vi "DeleteGraph2.vi"(10 "StileIn":T1(array[cluster])=[{"Plot.Bar Plot Style"=0, "Plot.DigitalLineStyle"=1, "Plot.Line Style"=0, "Plot.Line Width"=2, "Plot.Plot Color"=5863167, "Plot.Plot Name"="Plot 0", "Plot.Point Style"=0}, {"Plot.Bar Plot Style"=0, "Plot.DigitalLineStyle"=1, "Plot.Line Style"=0, "Plot.Line Width"=2, "Plot.Plot Color"=13257796, "Plot.Plot Name"="Plot 1", "Plot.Point Style"=0}, {"Plot.Bar Plot Style"=0, "Plot.DigitalLineStyle"=1, "Plot.Line Style"=0, "Plot.Line Width"=2, "Plot.Plot Color"=6601816, "Plot.Plot Name"="Plot 2", "Plot.Point Style"=0}, {"Plot.Bar Plot Style"=0, "Plot.DigitalLineStyle"=1, "Plot.Line Style"=0, "Plot.Line Width"=2, "Plot.Plot Color"=15441725, "Plot.Plot Name"="Plot 3", "Plot.Point Style"=0}, {"Plot.Bar Plot Style"=0, "Plot.DigitalLineStyle"=1, "Plot.Line Style"=0, "Plot.Line Width"=2, "Plot.Plot Color"=8742822, "Plot.Plot Name"="Plot 4", "Plot.Point Style"=0}, {"Plot.Bar Plot Style"=0, "Plot.DigitalLineStyle"=1, "Plot.Line Style"=0, "Plot.Line Width"=3, "Plot.Plot Color"=10051840, "Plot.Plot Name"="Plot 5", "Plot.Point Style"=0}, {"Plot.Bar Plot Style"=0, "Plot.DigitalLineStyle"=1, "Plot.Line Style"=0, "Plot.Line Width"=3, "Plot.Plot Color"=3121844, "Plot.Plot Name"="Plot 6", "Plot.Point Style"=0}, {"Plot.Bar Plot Style"=0, "Plot.DigitalLineStyle"=1, "Plot.Line Style"=0, "Plot.Line Width"=3, "Plot.Plot Color"=13592771, "Plot.Plot Name"="Plot 7", "Plot.Point Style"=0}, {"Plot.Bar Plot Style"=0, "Plot.DigitalLineStyle"=1, "Plot.Line Style"=0, "Plot.Line Width"=3, "Plot.Plot Color"=931427, "Plot.Plot Name"="Plot 8", "Plot.Point Style"=0}, {"Plot.Bar Plot Style"=0, "Plot.DigitalLineStyle"=1, "Plot.Line Style"=0, "Plot.Line Width"=3, "Plot.Plot Color"=9014678, "Plot.Plot Name"="Plot 9", "Plot.Point Style"=0}, {"Plot.Bar Plot Style"=0, "Plot.DigitalLineStyle"=1, "Plot.Line Style"=0, "Plot.Line Width"=0, "Plot.Plot Color"=14483242, "Plot.Plot Name"="Plot 10", "Plot.Point Style"=0}, {"Plot.Bar Plot Style"=0, "Plot.DigitalLineStyle"=1, "Plot.Line Style"=0, "Plot.Line Width"=1, "Plot.Plot Color"=9538739, "Plot.Plot Name"="Plot 11", "Plot.Point Style"=0}, {"Plot.Bar Plot Style"=0, "Plot.DigitalLineStyle"=1, "Plot.Line Style"=0, "Plot.Line Width"=0, "Plot.Plot Color"=982784, "Plot.Plot Name"="Plot 12", "Plot.Point Style"=0}, {"Plot.Bar Plot Style"=0, "Plot.DigitalLineStyle"=1, "Plot.Line Style"=0, "Plot.Line Width"=0, "Plot.Plot Color"=4375295, "Plot.Plot Name"="Plot 13", "Plot.Point Style"=0}, {"Plot.Bar Plot Style"=0, "Plot.DigitalLineStyle"=1, "Plot.Line Style"=0, "Plot.Line Width"=0, "Plot.Plot Color"=13827953, "Plot.Plot Name"="Plot 14", "Plot.Point Style"=0}, {"Plot.Bar Plot Style"=0, "Plot.DigitalLineStyle"=1, "Plot.Line Style"=0, "Plot.Line Width"=0, "Plot.Plot Color"=13457919, "Plot.Plot Name"="Plot 15", "Plot.Point Style"=0}, {"Plot.Bar Plot Style"=0, "Plot.DigitalLineStyle"=1, "Plot.Line Style"=0, "Plot.Line Width"=0, "Plot.Plot Color"=16757522, "Plot.Plot Name"="Plot 16", "Plot.Point Style"=0}, {"Plot.Bar Plot Style"=0, "Plot.DigitalLineStyle"=1, "Plot.Line Style"=0, "Plot.Line Width"=0, "Plot.Plot Color"=4343295, "Plot.Plot Name"="Plot 17", "Plot.Point Style"=0}, {"Plot.Bar Plot Style"=0, "Plot.DigitalLineStyle"=1, "Plot.Line Style"=0, "Plot.Line Width"=0, "Plot.Plot Color"=16728758, "Plot.Plot Name"="Plot 18", "Plot.Point Style"=0}, {"Plot.Bar Plot Style"=0, "Plot.DigitalLineStyle"=1, "Plot.Line Style"=0, "Plot.Line Width"=0, "Plot.Plot Color"=5898228, "Plot.Plot Name"="Plot 19", "Plot.Point Style"=0}], 11 "GraphIN":T2) -> (2 "StileOUT":T1(array[cluster]), 3 "GraphOUT":T2)   [LabVIEW 2017]
uses:
  controls/st_str Graph Data.ctl
  <vilib>/Utility/miscctls.llb/LVAnnotationListTypeDef.ctl
  <vilib>/Utility/miscctls.llb/LVCursorListTypeDef.ctl
panel:
  out "Array Stile 2":T1(array[cluster])
  out "x+y":dbl
  out "Array StileSave":T1(array[cluster])
  out "error out":errorcluster
  in  "DeleteALLPlot":bool
  out "Array Stile":T1(array[cluster])=[{"Plot.Bar Plot Style"=0, "Plot.DigitalLineStyle"=1, "Plot.Line Style"=0, "Plot.Line Width"=3, "Plot.Plot Color"=3113143, "Plot.Plot Name"=" Plot 0", "Plot.Point Style"=0}, {"Plot.Bar Plot Style"=0, "Plot.DigitalLineStyle"=1, "Plot.Line Style"=0, "Plot.Line Width"=3, "Plot.Plot Color"=13257796, "Plot.Plot Name"=" Plot 1", "Plot.Point Style"=0}, {"Plot.Bar Plot Style"=0, "Plot.DigitalLineStyle"=1, "Plot.Line Style"=0, "Plot.Line Width"=3, "Plot.Plot Color"=6601816, "Plot.Plot Name"="Plot 2", "Plot.Point Style"=0}, {"Plot.Bar Plot Style"=0, "Plot.DigitalLineStyle"=1, "Plot.Line Style"=0, "Plot.Line Width"=3, "Plot.Plot Color"=15441725, "Plot.Plot Name"="Plot 3", "Plot.Point Style"=0}, {"Plot.Bar Plot Style"=0, "Plot.DigitalLineStyle"=1, "Plot.Line Style"=0, "Plot.Line Width"=3, "Plot.Plot Color"=8742822, "Plot.Plot Name"="Plot 4", "Plot.Point Style"=0}, {"Plot.Bar Plot Style"=0, "Plot.DigitalLineStyle"=1, "Plot.Line Style"=0, "Plot.Line Width"=3, "Plot.Plot Color"=10051840, "Plot.Plot Name"="Plot 5", "Plot.Point Style"=0}, {"Plot.Bar Plot Style"=0, "Plot.DigitalLineStyle"=1, "Plot.Line Style"=0, "Plot.Line Width"=3, "Plot.Plot Color"=3121844, "Plot.Plot Name"="Plot 6", "Plot.Point Style"=0}, {"Plot.Bar Plot Style"=0, "Plot.DigitalLineStyle"=1, "Plot.Line Style"=0, "Plot.Line Width"=3, "Plot.Plot Color"=13592771, "Plot.Plot Name"="Plot 7", "Plot.Point Style"=0}, {"Plot.Bar Plot Style"=0, "Plot.DigitalLineStyle"=1, "Plot.Line Style"=0, "Plot.Line Width"=3, "Plot.Plot Color"=931427, "Plot.Plot Name"="Plot 8", "Plot.Point Style"=0}, {"Plot.Bar Plot Style"=0, "Plot.DigitalLineStyle"=1, "Plot.Line Style"=0, "Plot.Line Width"=3, "Plot.Plot Color"=9014678, "Plot.Plot Name"="Plot 9", "Plot.Point Style"=0}, {"Plot.Bar Plot Style"=0, "Plot.DigitalLineStyle"=1, "Plot.Line Style"=0, "Plot.Line Width"=0, "Plot.Plot Color"=16777215, "Plot.Plot Name"="Plot 10", "Plot.Point Style"=0}, {"Plot.Bar Plot Style"=0, "Plot.DigitalLineStyle"=1, "Plot.Line Style"=0, "Plot.Line Width"=0, "Plot.Plot Color"=16728642, "Plot.Plot Name"="Plot11", "Plot.Point Style"=0}, {"Plot.Bar Plot Style"=0, "Plot.DigitalLineStyle"=1, "Plot.Line Style"=0, "Plot.Line Width"=0, "Plot.Plot Color"=982784, "Plot.Plot Name"="Plot 12", "Plot.Point Style"=0}, {"Plot.Bar Plot Style"=0, "Plot.DigitalLineStyle"=1, "Plot.Line Style"=0, "Plot.Line Width"=0, "Plot.Plot Color"=4375295, "Plot.Plot Name"="Plot 13", "Plot.Point Style"=0}, {"Plot.Bar Plot Style"=0, "Plot.DigitalLineStyle"=1, "Plot.Line Style"=0, "Plot.Line Width"=0, "Plot.Plot Color"=13827953, "Plot.Plot Name"="Plot 14", "Plot.Point Style"=0}, {"Plot.Bar Plot Style"=0, "Plot.DigitalLineStyle"=1, "Plot.Line Style"=0, "Plot.Line Width"=0, "Plot.Plot Color"=13457919, "Plot.Plot Name"="Plot 15", "Plot.Point Style"=0}, {"Plot.Bar Plot Style"=0, "Plot.DigitalLineStyle"=1, "Plot.Line Style"=0, "Plot.Line Width"=0, "Plot.Plot Color"=16757522, "Plot.Plot Name"="Plot 16", "Plot.Point Style"=0}, {"Plot.Bar Plot Style"=0, "Plot.DigitalLineStyle"=1, "Plot.Line Style"=0, "Plot.Line Width"=0, "Plot.Plot Color"=4343295, "Plot.Plot Name"="Plot 17", "Plot.Point Style"=0}, {"Plot.Bar Plot Style"=0, "Plot.DigitalLineStyle"=1, "Plot.Line Style"=0, "Plot.Line Width"=0, "Plot.Plot Color"=16728758, "Plot.Plot Name"="Plot 18", "Plot.Point Style"=0}, {"Plot.Bar Plot Style"=0, "Plot.DigitalLineStyle"=1, "Plot.Line Style"=0, "Plot.Line Width"=0, "Plot.Plot Color"=5898228, "Plot.Plot Name"="Plot 19", "Plot.Point Style"=0}, {"Plot.Bar Plot Style"=0, "Plot.DigitalLineStyle"=1, "Plot.Line Style"=0, "Plot.Line Width"=3, "Plot.Plot Color"=476624, "Plot.Plot Name"="Plot 20", "Plot.Point Style"=0}, {"Plot.Bar Plot Style"=0, "Plot.DigitalLineStyle"=1, "Plot.Line Style"=0, "Plot.Line Width"=3, "Plot.Plot Color"=411336, "Plot.Plot Name"="Plot 21", "Plot.Point Style"=0}]
  in  "DeleteSelectPlot":bool
  in  "Exit":bool
  out "АЧХIn":cluster{dbl[], dbl[]}[](graph)=[{[10.0], [0.9990420594251289]}, {[10.0, 20.0, 30.0, 40.0, 50.0, 60.0, 70.0, 80.0, 90.0, 100.0], [0.9990710865943554, 0.9983737368547715, 0.9976213766215998, 0.9969952678672057, 0.9967386681898875, 0.9967158758213325, 0.9966216633883461, 0.9967130281386235, 0.997241304832117, 0.9978171905888101]}, {[10.0, 20.0, 30.0, 40.0, 50.0, 60.0, 70.0, 80.0, 90.0, 100.0], [0.9988829040935796, 0.998316804468434, 0.9975357463328959, 0.9968238922918776, 0.9966331250389342, 0.9964782615048055, 0.9964769254923784, 0.9965780617245455, 0.9971895145348859, 0.9977820844166819]}, {[100.0, 110.0, 120.0, 130.0, 140.0, 150.0, 160.0, 170.0, 180.0, 190.0, 200.0], [0.9976024425934543, 0.9979153955951243, 0.9977501265851223, 0.9976091903479634, 0.997569296017074, 0.9976312638585361, 0.9976378149884235, 0.9975972662804196, 0.9976213719667596, 0.9977412021645674, 0.9978437042833532]}] caption="XY Graph - Light"
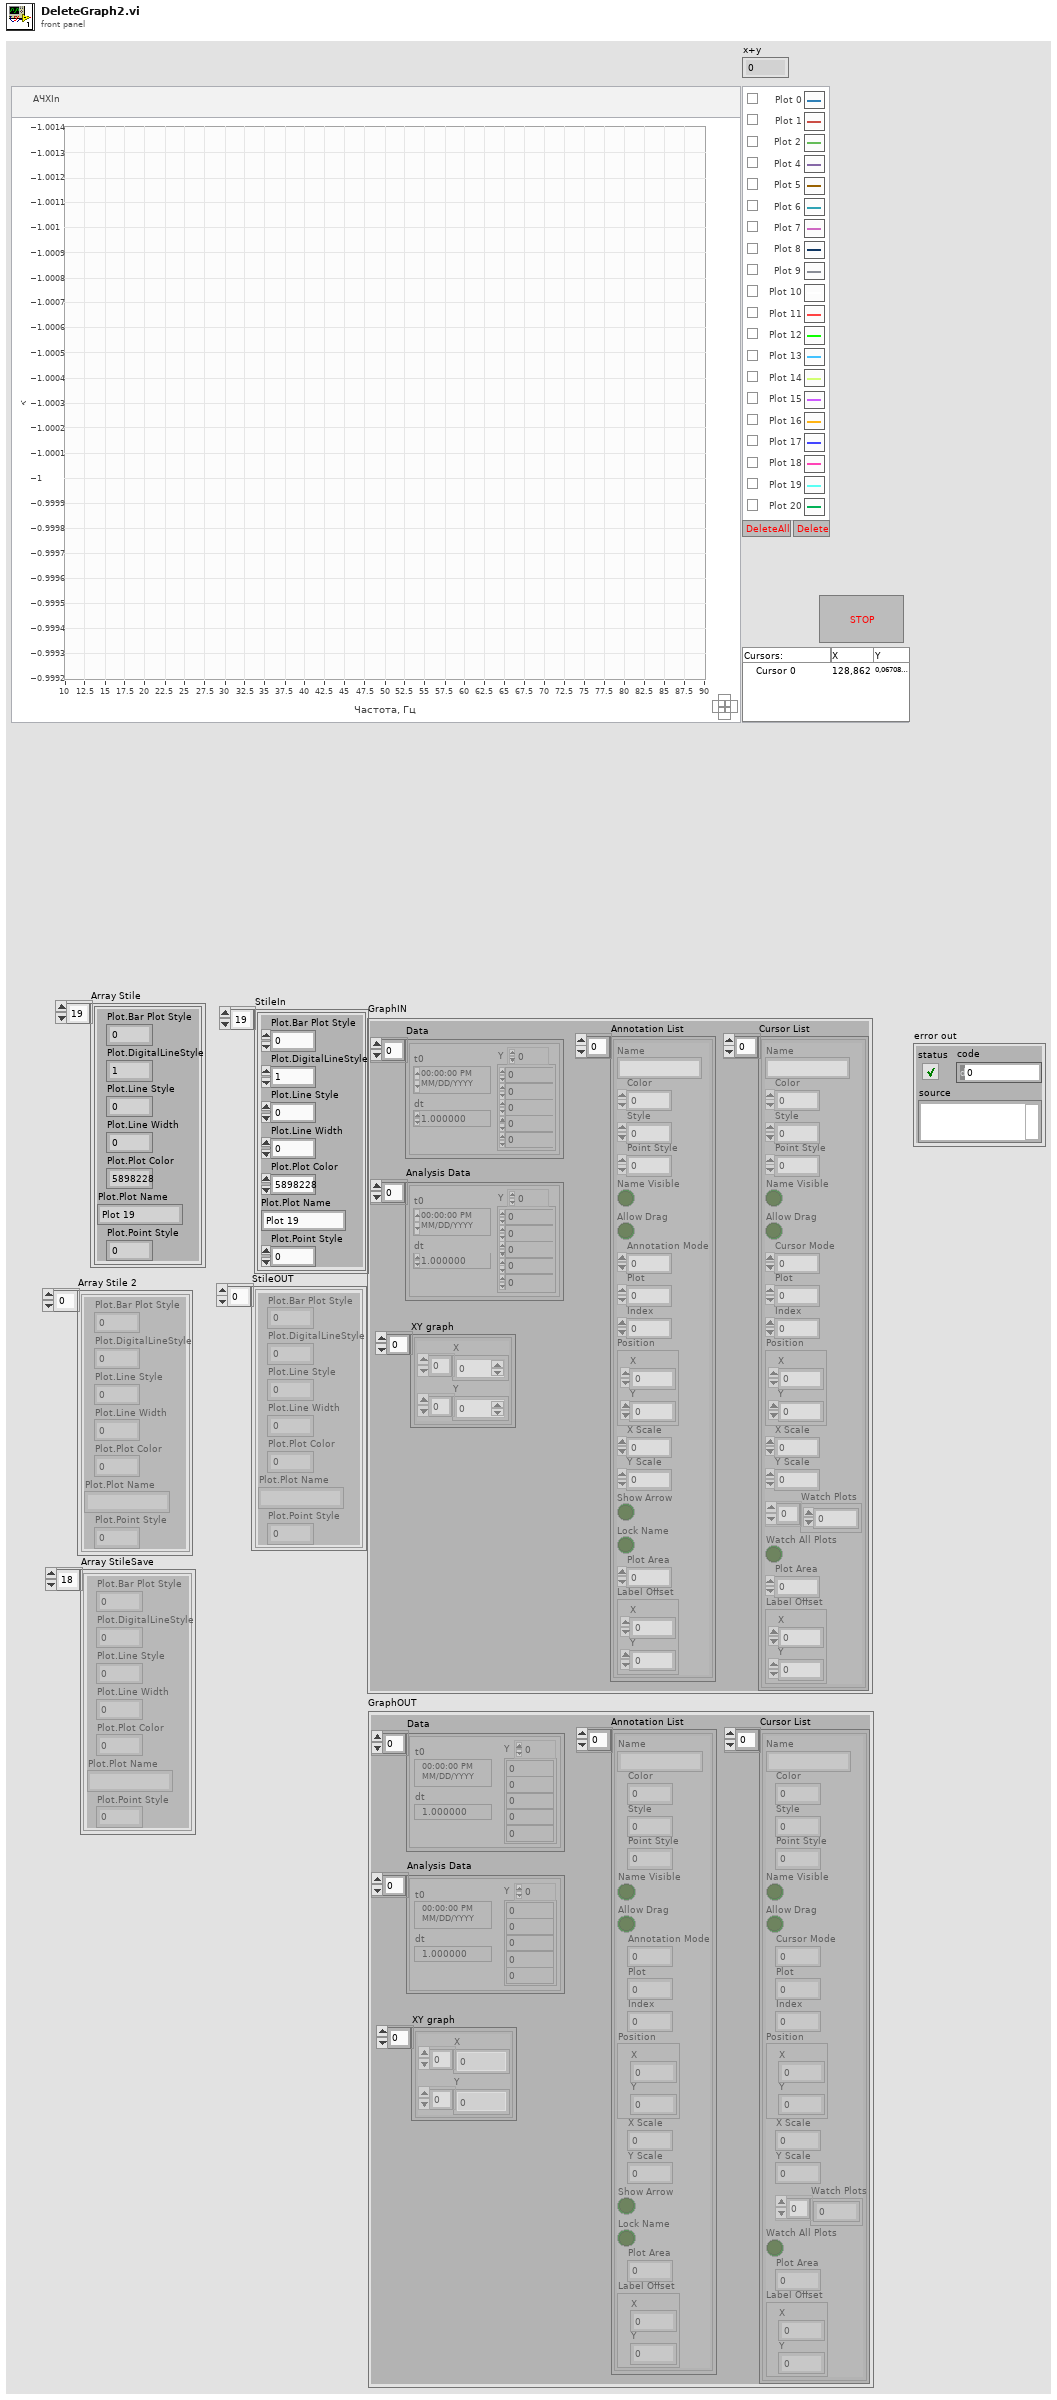
[diagram p1: front panel]
types:
  T1 = cluster{"Plot.Bar Plot Style":u8, "Plot.DigitalLineStyle":u8, "Plot.Line Style":u8, "Plot.Line Width":u8, "Plot.Plot Color":u32, "Plot.Plot Name":string, "Plot.Point Style":u8}[]
  T2 = typedef "st_str Graph Data.ctl" = cluster{"Data":waveform(dbl)[], "Annotation List":T3, "Cursor List":T4, "Analysis Data":waveform(dbl)[], "XY graph":cluster{"X":dbl[], "Y":dbl[]}[]}
  T3 = typedef "LVAnnotationListTypeDef.ctl" = cluster{"Name":string, "Color":u32, "Style":u8, "Point Style":u8, "Name Visible":bool, "Allow Drag":bool, "Annotation Mode":u32, "Plot":i32, "Index":i32, "Position":cluster{"X":dbl, "Y":dbl}, "X Scale":u32, "Y Scale":u32, "Show Arrow":bool, "Lock Name":bool, "Plot Area":i32, "Label Offset":cluster{"X":dbl, "Y":dbl}}[]
  T4 = typedef "LVCursorListTypeDef.ctl" = cluster{"Name":string, "Color":u32, "Style":u8, "Point Style":u8, "Name Visible":bool, "Allow Drag":bool, "Cursor Mode":u32, "Plot":i32, "Index":i32, "Position":cluster{"X":dbl, "Y":dbl}, "X Scale":u32, "Y Scale":u32, "Watch Plots":i32[], "Watch All Plots":bool, "Plot Area":i32, "Label Offset":cluster{"X":dbl, "Y":dbl}}[]
  T5 = cluster{"Plot.Bar Plot Style":u8, "Plot.DigitalLineStyle":u8, "Plot.Line Style":u8, "Plot.Line Width":u8, "Plot.Plot Color":u32, "Plot.Plot Name":string, "Plot.Point Style":u8}
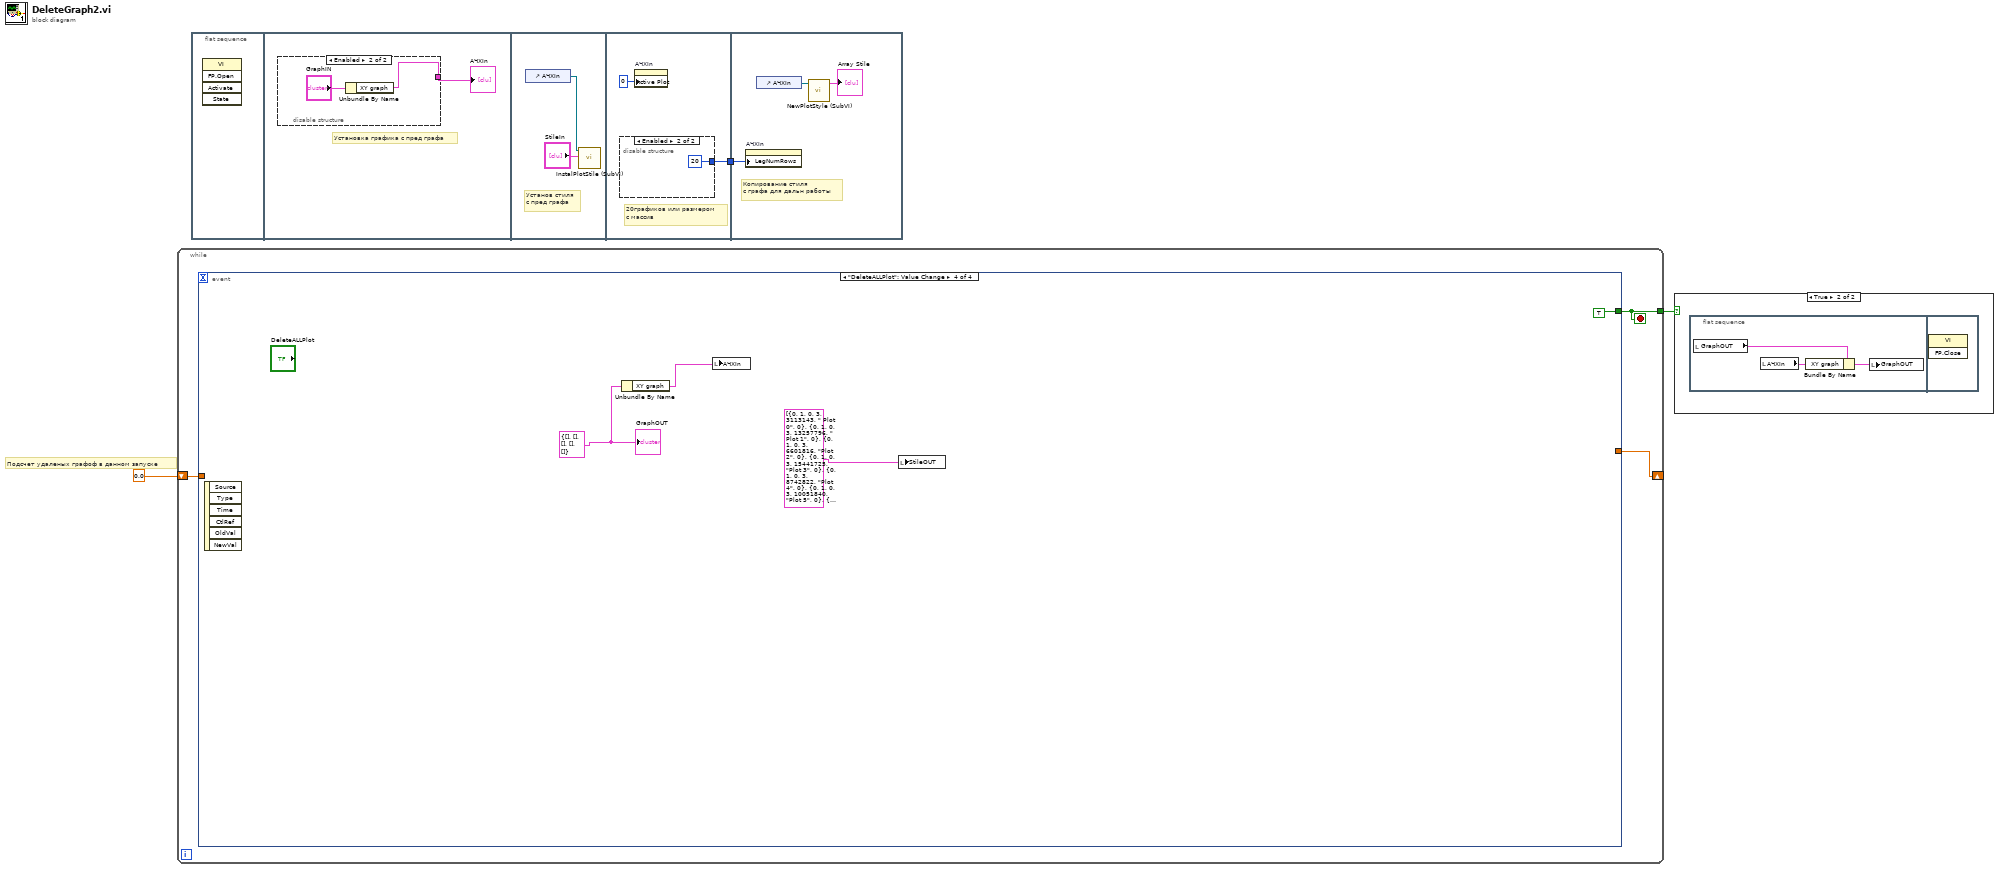
[diagram p0: block diagram]
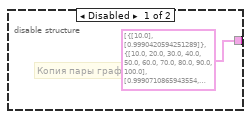
[diagram p3: hidden frame]
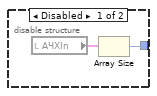
[diagram p4: hidden frame]
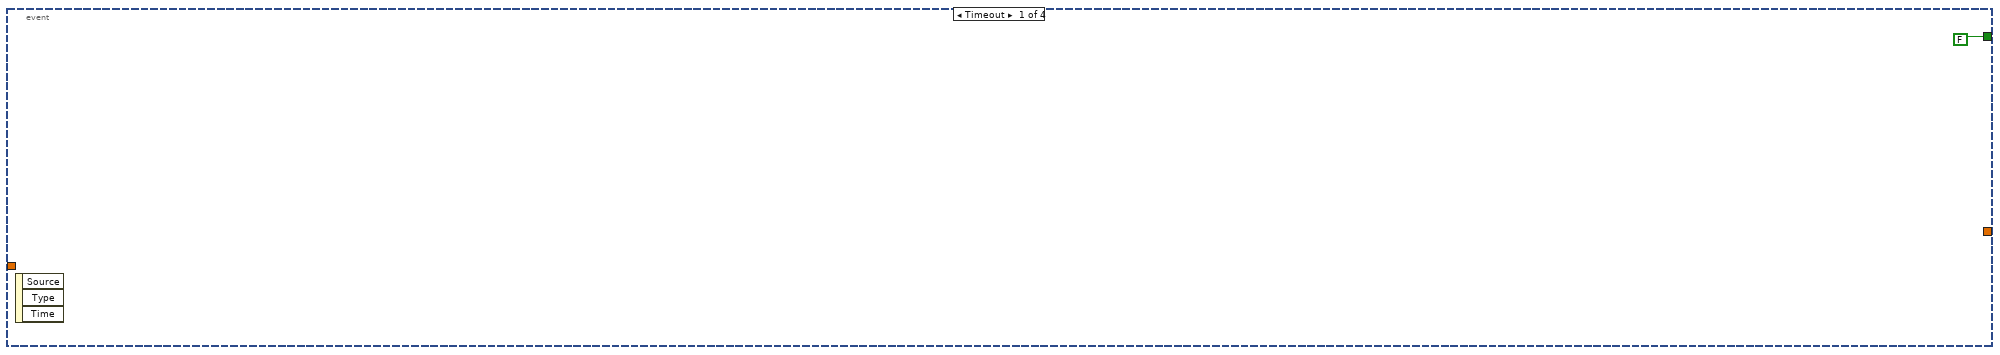
[diagram p5: hidden frame]
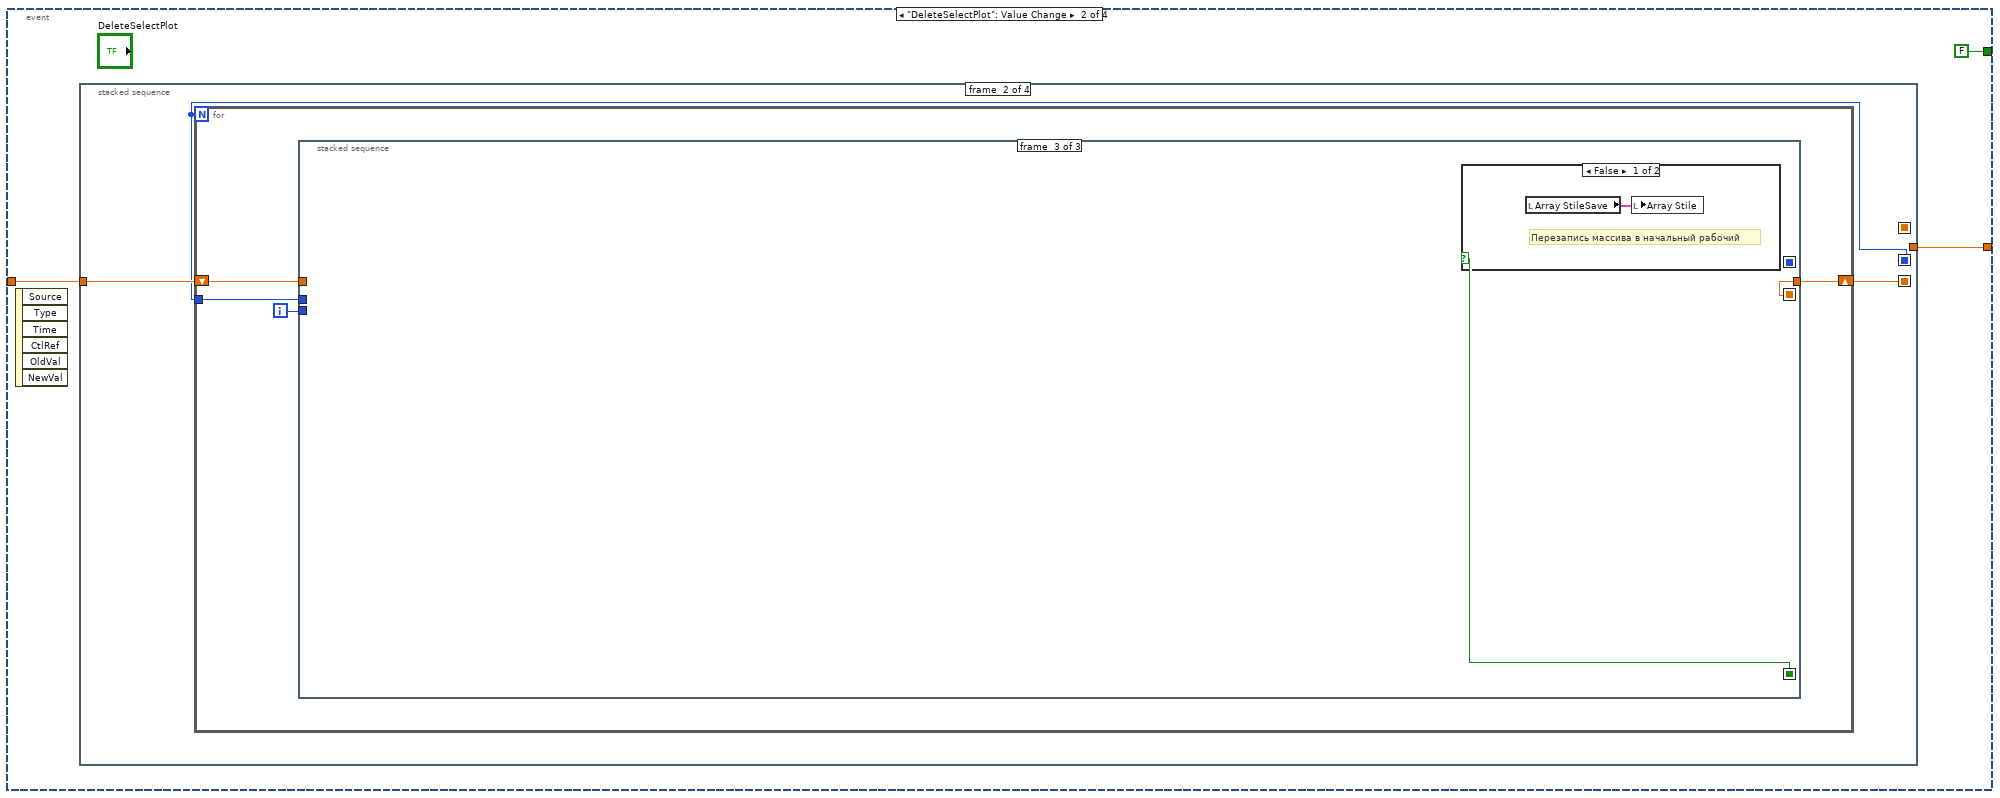
[diagram p6: hidden frame]
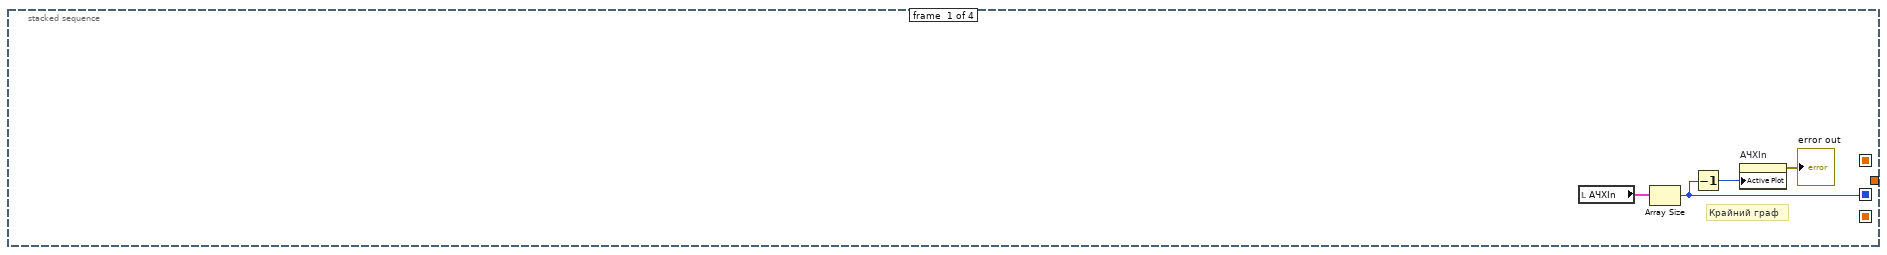
[diagram p7: hidden frame]
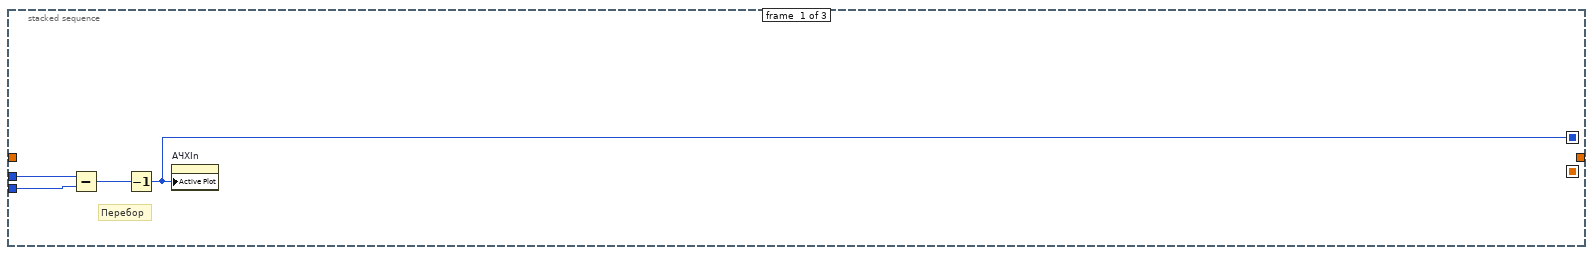
[diagram p8: hidden frame]
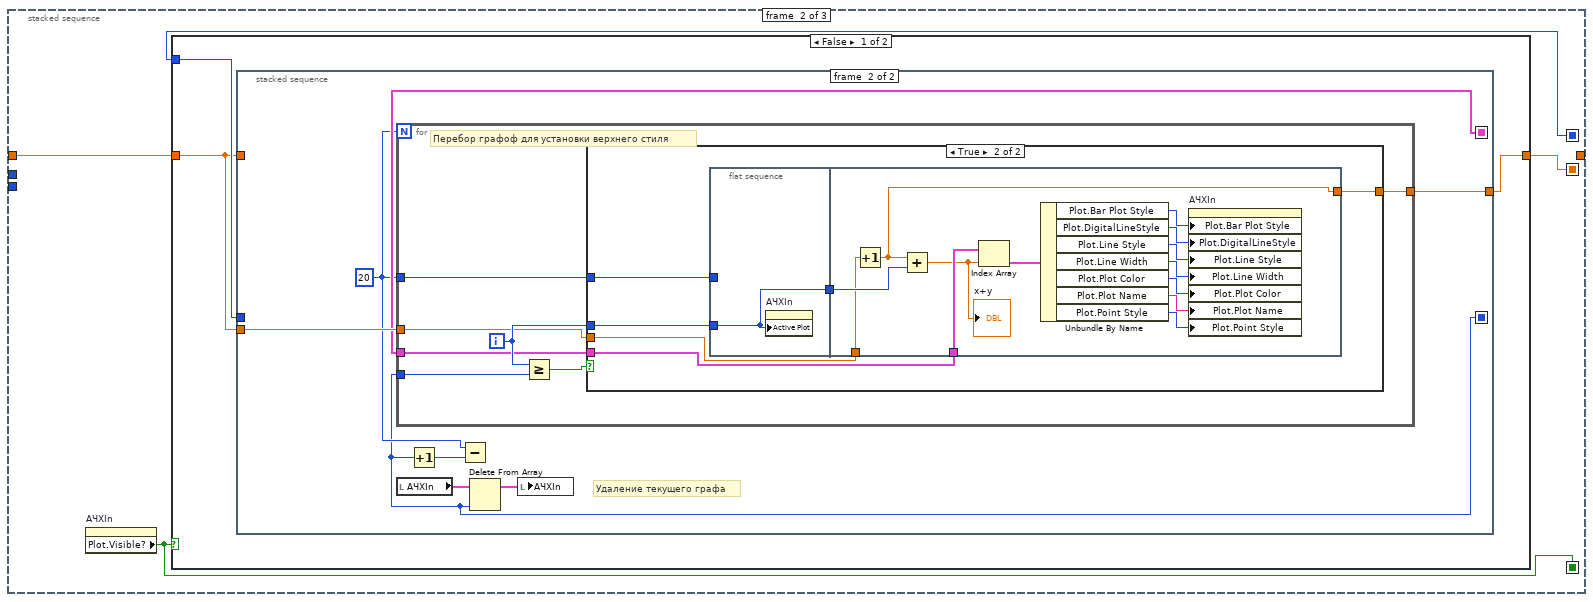
[diagram p9: hidden frame]
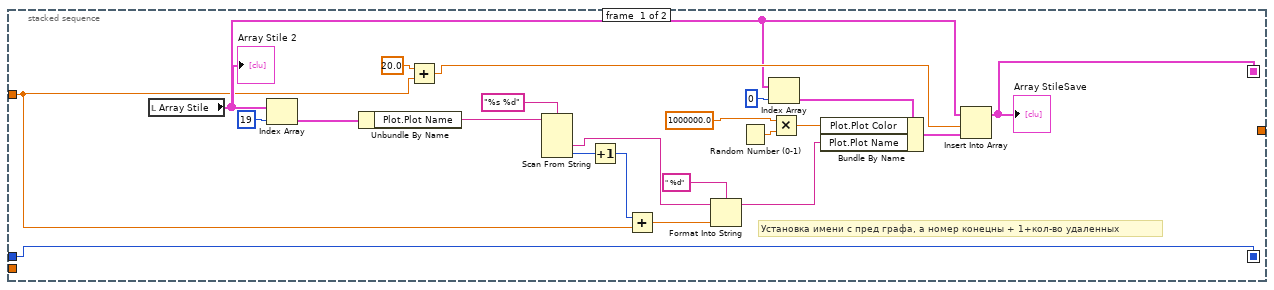
[diagram p10: hidden frame]
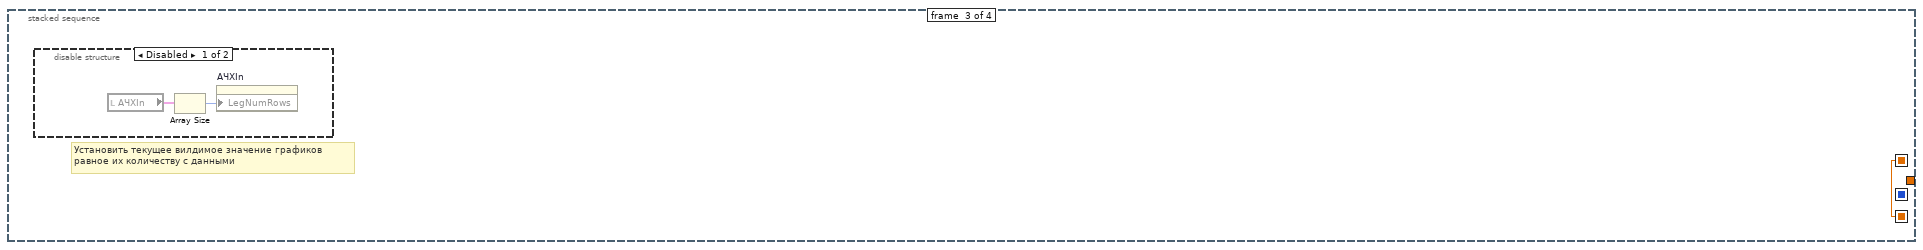
[diagram p14: hidden frame]
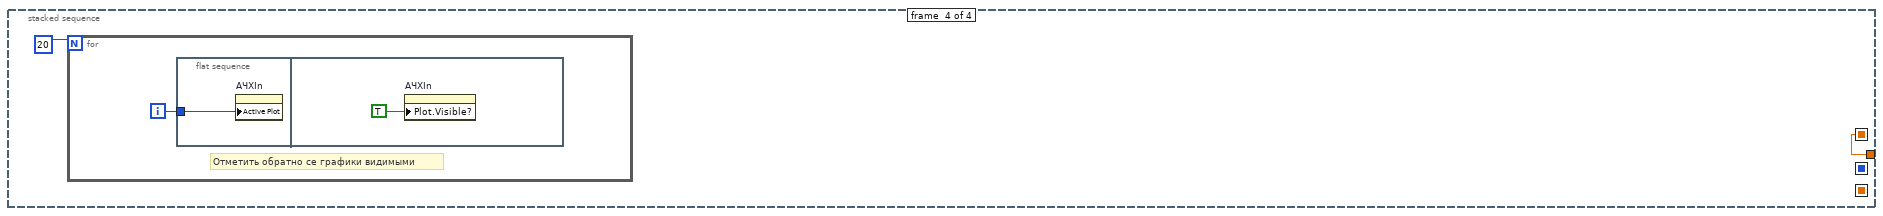
[diagram p16: hidden frame]
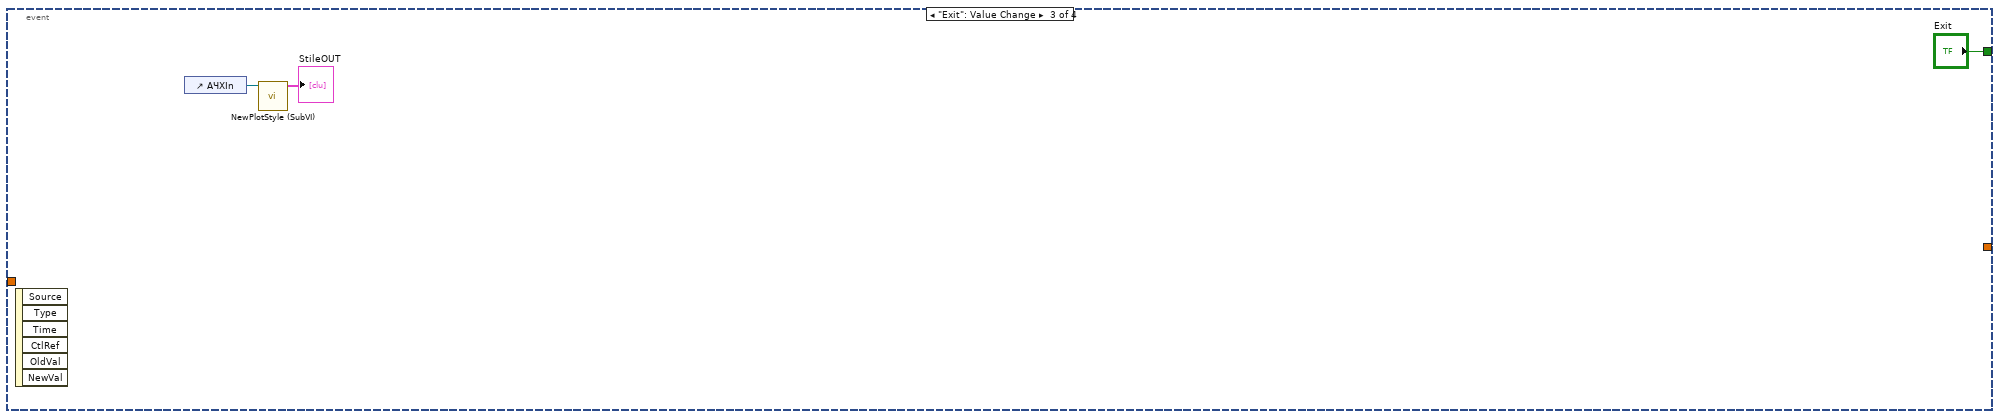
[diagram p17: hidden frame]
diagram:
  # "Подсчет удаленых графоф в данном запуске"
  n1 = while {
    shift-right: [w6] -> _
    shift-left: 0.0 -> [w5]
    tunnel: [w4] -> w1
    stop <- w4 stop-if-true
    n2 = event shown="[3] \"DeleteALLPlot\": Value Change" {
      selector: _ -> [_ _ _ _]
      dyn-events: _ -> [_ _ _ _]
      timeout: _ -> [_ _ _ _]
      tunnel: [_ w10 _ _] -> w6
      tunnel: w5 -> [_ w9 _ _]
      tunnel: [FALSE ("Exit") FALSE ("Exit") "Exit" TRUE ("Exit")] -> w4
      event Timeout {
        n3 = event-data() -> ()  [unwired: 1 in, 3 out]
      }
      event "DeleteSelectPlot": Value Change {
        n4 = event-data() -> ()  [unwired: 1 in, 6 out]
        n5 = stacked-sequence {
          seq-local: [w12 _ _ _] -> [_ w16 _ _]
          seq-local: [_ w15 _ _] -> [_ _ w95 _]
          seq-local: [_ _ w95 _] -> [_ _ _ w99]
          tunnel: w9 -> [_ w17 _ _]
          tunnel: [_ _ _ w99] -> w10
          frame #0 {
            # "Крайний граф"
            n6 = local read "АЧХIn"() -> (w14:cluster{dbl[], dbl[]}[])
            n7 = Array Size(array=w14) -> (size(s)=w12:i32)
            n8 = Decrement(x=w12) -> (x-1=w13:i32)
            n9 = property on="АЧХIn" class="XYGraph (strict)"("Active Plot"=w13) -> (error out=→"error out":errorcluster)  [unwired: 2 in, 1 out]
          }
          frame #1 {
            n10 = for {
              N: w16 -> [_]
              tunnel: w16 -> [w20]
              shift-right: [w18] -> w15
              shift-left: w17 -> [w19]
              i -> [w21]
              n11 = stacked-sequence {
                seq-local: [w22 _ _] -> [_ w29 _]
                seq-local: [_ w28 _] -> [_ _ w93]
                seq-local: [_ w26 _] -> [_ _ w92]
                tunnel: w21 -> [w25 _ _]
                tunnel: w20 -> [w24 _ _]
                tunnel: w19 -> [_ w27 _]
                tunnel: [_ _ w93] -> w18
                frame #0 {
                  # "Перебор"
                  n12 = Subtract(x=w24, y=w25) -> (x-y=w23:i32)
                  n13 = Decrement(x=w23) -> (x-1=w22:i32)
                  n14 = property on="АЧХIn" class="XYGraph (strict)"("Active Plot"=w22) -> ()  [unwired: 2 in, 2 out]
                }
                frame #1 {
                  n15 = property on="АЧХIn" class="XYGraph (strict)"() -> ("Plot.Visible?"=w26:bool)  [unwired: 2 in, 2 out]
                  n16 = case shown="False" w26 {
                    tunnel: w29 -> [w32 _]
                    tunnel: [w31 w91] -> w28
                    tunnel: w27 -> [w30 w91]
                    frame False {
                      n17 = stacked-sequence {
                        seq-local: [w54 _] -> [_ w55]
                        seq-local: [w34 _] -> [_ w58]
                        tunnel: w32 -> [w54 _]
                        tunnel: w30 -> [w38 _]
                        tunnel: w30 -> [_ w59]
                        tunnel: [_ w60] -> w31
                        frame #0 {
                          # "Установка имени с пред графа, а номер конецны + 1+кол-во удаленных"
                          n18 = local read "Array Stile"() -> (w43:T1)
                          "Array Stile 2" <- w43
                          n19 = Index Array(array=w43, index=19) -> (element=w42:T5)
                          n20 = Unbundle By Name(w42) -> ("Plot.Plot Name"=w41:string)
                          n21 = Add(x=20.0, y=w38) -> (x+y=w52:dbl)
                          n22 = Scan From String(format string="%s %d", input string=w41) -> (output 1=w33:string, output 2=w36:i32)  [unwired: 4 in, 3 out]
                          n23 = Increment(x=w36) -> (x+1=w35:i32)
                          n24 = Add(x=w35, y=w38) -> (x+y=w37:dbl)
                          n25 = Format Into String(format string=" %d", initial string=w33, w37) -> (resulting string=w49:string)  [unwired: 1 in, 1 out]
                          n26 = Random Number (0-1)() -> (number: 0 to 1=w48:dbl)
                          n27 = Index Array(array=w43, index=0) -> (element=w50:T5)
                          n28 = Multiply(x=1000000.0, y=w48) -> (x*y=w46:dbl)
                          n29 = Bundle By Name(cluster=w50, "Plot.Plot Color"=w46, "Plot.Plot Name"=w49) -> (w45:T5)
                          n30 = Insert Into Array(array=w43, index=w52, new element=w45) -> (w34:T1)
                          "Array StileSave" <- w34
                        }
                        frame #1 {
                          w57 = 20
                          # "Удаление текущего графа"
                          n31 = for {
                            N: w57 -> [_]
                            tunnel: w55 -> [w66]
                            tunnel: w58 -> [w68]
                            tunnel: w57 -> [w67]
                            tunnel: [w64] -> w60
                            tunnel: w59 -> [w63]
                            i -> [w69]
                            # "Перебор графоф для установки верхнего стиля"
                            n32 = Greater Or Equal?(x=w69, y=w66) -> (x >= y?=w65:bool)
                            n33 = case shown="True" w65 {
                              tunnel: w69 -> [_ w76]
                              tunnel: w68 -> [_ w75]
                              tunnel: [w70 w73] -> w64
                              tunnel: w67 -> [_ w72]
                              tunnel: w63 -> [w70 w71]
                              frame False {
                              }
                              frame True {
                                n34 = flat-sequence {
                                tunnel: w76 -> [w77]
                                tunnel: [w77] -> w74
                                tunnel: w72 -> [_]
                                tunnel: w75 -> [w83]
                                tunnel: w74 -> [w81]
                                tunnel: [w78] -> w73
                                tunnel: w71 -> [w79]
                                frame #0 {
                                n35 = property on="АЧХIn" class="XYGraph (strict)"("Active Plot"=w77) -> ()  [unwired: 2 in, 2 out]
                                }
                                frame #1 {
                                n36 = Increment(x=w79) -> (x+1=w78:dbl)
                                n37 = Add(x=w78, y=w81) -> (x+y=w80:dbl)
                                "x+y" <- w80
                                n38 = Index Array(array=w83, index=w80) -> (element=w82:T5)
                                n39 = Unbundle By Name(w82) -> ("Plot.Bar Plot Style"=w90:u8, "Plot.DigitalLineStyle"=w89:u8, "Plot.Line Style"=w88:u8, "Plot.Line Width"=w87:u8, "Plot.Plot Color"=w86:u32, "Plot.Plot Name"=w85:string, "Plot.Point Style"=w84:u8)
                                n40 = property on="АЧХIn" class="XYGraph (strict)"("Plot.Bar Plot Style"=w90, "Plot.DigitalLineStyle"=w89, "Plot.Line Style"=w88, "Plot.Line Width"=w87, "Plot.Plot Color"=w86, "Plot.Plot Name"=w85, "Plot.Point Style"=w84) -> ()  [unwired: 2 in, 2 out]
                                }
                                }
                              }
                            }
                          }
                          n41 = local read "АЧХIn"() -> (w62:cluster{dbl[], dbl[]}[])
                          n42 = Increment(x=w55) -> (x+1=w56:i32)
                          n43 = Subtract(x=w57, y=w56) -> ()  [unwired: 1 out]
                          n44 = Delete From Array(array=w62, index=w55) -> (array with subset deleted=w61:cluster{dbl[], dbl[]}[])  [unwired: 1 in, 1 out]
                          n45 = local write "АЧХIn"(w61) -> ()
                        }
                      }
                    }
                    frame True {
                    }
                  }
                }
                frame #2 {
                  n46 = case shown="False" w92 {
                    frame False {
                      # "Перезапись массива в начальный рабочий"
                      n47 = local read "Array StileSave"() -> (w94:T1)
                      n48 = local write "Array Stile"(w94) -> ()
                    }
                    frame True {
                    }
                  }
                }
              }
            }
          }
          frame #2 {
            # "Установить текущее вилдимое значение графиков\nравное их количеству с данными"
            n49 = disable-structure shown="Disabled" {
              frame Disabled {
                n50 = local read "АЧХIn"() -> (w96:cluster{dbl[], dbl[]}[])
                n51 = Array Size(array=w96) -> (size(s)=w97:i32)
                n52 = property on="АЧХIn" class="XYGraph (strict)"("LegNumRows"=w97) -> ()  [unwired: 2 in, 2 out]
              }
              frame Enabled {
              }
            }
          }
          frame #3 {
            n53 = for {
              N: 20 -> [_]
              i -> [w100]
              # "Отметить обратно се графики видимыми"
              n54 = flat-sequence {
                tunnel: w100 -> [w101]
                frame #0 {
                  n55 = property on="АЧХIn" class="XYGraph (strict)"("Active Plot"=w101) -> ()  [unwired: 2 in, 2 out]
                }
                frame #1 {
                  n56 = property on="АЧХIn" class="XYGraph (strict)"("Plot.Visible?"=TRUE ("Plot.Visible")) -> ()  [unwired: 2 in, 2 out]
                }
              }
            }
          }
        }
      }
      event "Exit": Value Change {
        n57 = event-data() -> ()  [unwired: 1 in, 6 out]
        n58 = control-ref of="АЧХIn"() -> (w104:refnum<vi>)
        n59 = call "NewPlotStyle (SubVI).vi"("XYGraph in"=w104) -> ("Array"=→"StileOUT":T1)  [unwired: 10 in]
      }
      event "DeleteALLPlot": Value Change {
        w107 = T2 {"Data"=[], "Annotation List"=[], "Cursor List"=[], "Analysis Data"=[], "XY graph"=[]} ("ClearGraph")
        n60 = event-data() -> ()  [unwired: 1 in, 6 out]
        n61 = Unbundle By Name(w107) -> ("XY graph"=w106:cluster{"X":dbl[], "Y":dbl[]}[])
        n62 = local write "АЧХIn"(w106) -> ()
        n63 = local write "StileOUT"(T1 [{"Plot.Bar Plot Style"=0, "Plot.DigitalLineStyle"=1, "Plot.Line Style"=0, "Plot.Line Width"=3, "Plot.Plot Color"=3113143, "Plot.Plot Name"=" Plot 0", "Plot.Point Style"=0}, {"Plot.Bar Plot Style"=0, "Plot.DigitalLineStyle"=1, "Plot.Line Style"=0, "Plot.Line Width"=3, "Plot.Plot Color"=13257796, "Plot.Plot Name"=" Plot 1", "Plot.Point Style"=0}, {"Plot.Bar Plot Style"=0, "Plot.DigitalLineStyle"=1, "Plot.Line Style"=0, "Plot.Line Width"=3, "Plot.Plot Color"=6601816, "Plot.Plot Name"="Plot 2", "Plot.Point Style"=0}, {"Plot.Bar Plot Style"=0, "Plot.DigitalLineStyle"=1, "Plot.Line Style"=0, "Plot.Line Width"=3, "Plot.Plot Color"=15441725, "Plot.Plot Name"="Plot 3", "Plot.Point Style"=0}, {"Plot.Bar Plot Style"=0, "Plot.DigitalLineStyle"=1, "Plot.Line Style"=0, "Plot.Line Width"=3, "Plot.Plot Color"=8742822, "Plot.Plot Name"="Plot 4", "Plot.Point Style"=0}, {"Plot.Bar Plot Style"=0, "Plot.DigitalLineStyle"=1, "Plot.Line Style"=0, "Plot.Line Width"=3, "Plot.Plot Color"=10051840, "Plot.Plot Name"="Plot 5", "Plot.Point Style"=0}, {"Plot.Bar Plot Style"=0, "Plot.DigitalLineStyle"=1, "Plot.Line Style"=0, "Plot.Line Width"=3, "Plot.Plot Color"=3121844, "Plot.Plot Name"="Plot 6", "Plot.Point Style"=0}, {"Plot.Bar Plot Style"=0, "Plot.DigitalLineStyle"=1, "Plot.Line Style"=0, "Plot.Line Width"=3, "Plot.Plot Color"=13592771, "Plot.Plot Name"="Plot 7", "Plot.Point Style"=0}, {"Plot.Bar Plot Style"=0, "Plot.DigitalLineStyle"=1, "Plot.Line Style"=0, "Plot.Line Width"=3, "Plot.Plot Color"=931427, "Plot.Plot Name"="Plot 8", "Plot.Point Style"=0}, {"Plot.Bar Plot Style"=0, "Plot.DigitalLineStyle"=1, "Plot.Line Style"=0, "Plot.Line Width"=3, "Plot.Plot Color"=9014678, "Plot.Plot Name"="Plot 9", "Plot.Point Style"=0}, {"Plot.Bar Plot Style"=0, "Plot.DigitalLineStyle"=1, "Plot.Line Style"=0, "Plot.Line Width"=0, "Plot.Plot Color"=16777215, "Plot.Plot Name"="Plot 10", "Plot.Point Style"=0}, {"Plot.Bar Plot Style"=0, "Plot.DigitalLineStyle"=1, "Plot.Line Style"=0, "Plot.Line Width"=0, "Plot.Plot Color"=16728642, "Plot.Plot Name"="Plot11", "Plot.Point Style"=0}, {"Plot.Bar Plot Style"=0, "Plot.DigitalLineStyle"=1, "Plot.Line Style"=0, "Plot.Line Width"=0, "Plot.Plot Color"=982784, "Plot.Plot Name"="Plot 12", "Plot.Point Style"=0}, {"Plot.Bar Plot Style"=0, "Plot.DigitalLineStyle"=1, "Plot.Line Style"=0, "Plot.Line Width"=0, "Plot.Plot Color"=4375295, "Plot.Plot Name"="Plot 13", "Plot.Point Style"=0}, {"Plot.Bar Plot Style"=0, "Plot.DigitalLineStyle"=1, "Plot.Line Style"=0, "Plot.Line Width"=0, "Plot.Plot Color"=13827953, "Plot.Plot Name"="Plot 14", "Plot.Point Style"=0}, {"Plot.Bar Plot Style"=0, "Plot.DigitalLineStyle"=1, "Plot.Line Style"=0, "Plot.Line Width"=0, "Plot.Plot Color"=13457919, "Plot.Plot Name"="Plot 15", "Plot.Point Style"=0}, {"Plot.Bar Plot Style"=0, "Plot.DigitalLineStyle"=1, "Plot.Line Style"=0, "Plot.Line Width"=0, "Plot.Plot Color"=16757522, "Plot.Plot Name"="Plot 16", "Plot.Point Style"=0}, {"Plot.Bar Plot Style"=0, "Plot.DigitalLineStyle"=1, "Plot.Line Style"=0, "Plot.Line Width"=0, "Plot.Plot Color"=4343295, "Plot.Plot Name"="Plot 17", "Plot.Point Style"=0}, {"Plot.Bar Plot Style"=0, "Plot.DigitalLineStyle"=1, "Plot.Line Style"=0, "Plot.Line Width"=0, "Plot.Plot Color"=16728758, "Plot.Plot Name"="Plot 18", "Plot.Point Style"=0}, {"Plot.Bar Plot Style"=0, "Plot.DigitalLineStyle"=1, "Plot.Line Style"=0, "Plot.Line Width"=0, "Plot.Plot Color"=5898228, "Plot.Plot Name"="Plot 19", "Plot.Point Style"=0}] ("Array")) -> ()
        "GraphOUT" <- w107
      }
    }
  }
  n64 = flat-sequence {
    tunnel: [w116] -> w3
    tunnel: w3 -> [w123]
    frame #0 {
      n65 = invoke class="VI" method="FP.Open"() -> ()  [unwired: 5 in, 5 out]
    }
    frame #1 {
      # "Установка графика с пред графа"
      n66 = disable-structure shown="Enabled" {
        disable-tunnel: [cluster{dbl[], dbl[]}[] [{[10.0], [0.9990420594251289]}, {[10.0, 20.0, 30.0, 40.0, 50.0, 60.0, 70.0, 80.0, 90.0, 100.0], [0.9990710865943554, 0.9983737368547715, 0.9976213766215998, 0.9969952678672057, 0.9967386681898875, 0.9967158758213325, 0.9966216633883461, 0.9967130281386235, 0.997241304832117, 0.9978171905888101]}, {[10.0, 20.0, 30.0, 40.0, 50.0, 60.0, 70.0, 80.0, 90.0, 100.0], [0.9988829040935796, 0.998316804468434, 0.9975357463328959, 0.9968238922918776, 0.9966331250389342, 0.9964782615048055, 0.9964769254923784, 0.9965780617245455, 0.9971895145348859, 0.9977820844166819]}, {[100.0, 110.0, 120.0, 130.0, 140.0, 150.0, 160.0, 170.0, 180.0, 190.0, 200.0], [0.9976024425934543, 0.9979153955951243, 0.9977501265851223, 0.9976091903479634, 0.997569296017074, 0.9976312638585361, 0.9976378149884235, 0.9975972662804196, 0.9976213719667596, 0.9977412021645674, 0.9978437042833532]}] ("АЧХ") w112] -> w110
        frame Disabled {
          # "Копия пары графиков"
        }
        frame Enabled {
          n67 = Unbundle By Name("GraphIN") -> ("XY graph"=w112:cluster{"X":dbl[], "Y":dbl[]}[])
        }
      }
      "АЧХIn" <- w110
    }
    frame #2 {
      # "Установ стиля\nс пред графа"
      n68 = control-ref of="АЧХIn"() -> (w114:refnum<vi>)
      n69 = call "InstalPlotStile (SubVI).vi"("StileIn"="StileIn", "XYGraph in"=w114) -> ()  [unwired: 10 in]
    }
    frame #3 {
      # "20графиков или размером\nс массив"
      n70 = disable-structure shown="Enabled" {
        disable-tunnel: [w119 20] -> w116
        frame Disabled {
          n71 = local read "АЧХIn"() -> (w118:cluster{dbl[], dbl[]}[])
          n72 = Array Size(array=w118) -> (size(s)=w119:i32)
        }
        frame Enabled {
        }
      }
      n73 = property on="АЧХIn" class="XYGraph (strict)"("Active Plot"=u32 0) -> ()  [unwired: 2 in, 2 out]
    }
    frame #4 {
      # "Копирование стиля \nс графа для дальн работы"
      n74 = property on="АЧХIn" class="XYGraph (strict)"("LegNumRows"=w123) -> ()  [unwired: 2 in, 2 out]
      n75 = control-ref of="АЧХIn"() -> (w122:refnum<vi>)
      n76 = call "NewPlotStyle (SubVI).vi"("XYGraph in"=w122) -> ("Array"=→"Array Stile":T1)  [unwired: 10 in]
    }
  }
  n77 = case shown="True" w1 {
    frame False {
    }
    frame True {
      n78 = flat-sequence {
        frame #0 {
          n79 = local read "GraphOUT"() -> (w126:T2)
          n80 = local read "АЧХIn"() -> (w124:cluster{dbl[], dbl[]}[])
          n81 = Bundle By Name(cluster=w126, "XY graph"=w124) -> (w125:T2)
          n82 = local write "GraphOUT"(w125) -> ()
        }
        frame #1 {
          n83 = invoke class="VI" method="FP.Close"() -> ()  [unwired: 3 in, 3 out]
        }
      }
    }
  }
